vi "advertise.vi"(10 "type":string, 11 "topic":string) -> (3 "JSON string":string)   [LabVIEW 2014]
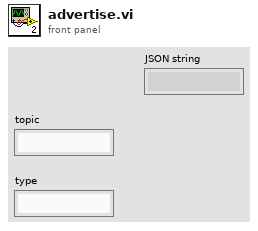
[diagram p1: front panel]
types:
  T1 = cluster{"op":string, "topic":string, "type":string}
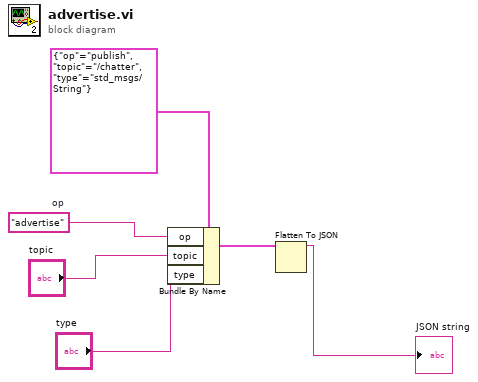
[diagram p0: block diagram]
diagram:
  w2 = "advertise"  # op
  n1 = Bundle By Name(cluster=T1 {"op"="publish", "topic"="/chatter", "type"="std_msgs/String"}, "op"=w2, "topic"="topic", "type"="type") -> (w5:T1)
  n2 = Flatten To JSON(anything=w5) -> (JSON string=→"JSON string":string)  [unwired: 2 in, 1 out]
